vi "from string.vi"(8 "error in":errorcluster, 9 "data":string, 10 "version":string, 11 "Missing Plugin configuration in":refnum<class "Missing Plugin configuration.lvclass">) -> (0 "error out":errorcluster, 3 "Missing Plugin configuration out":refnum<class "Missing Plugin configuration.lvclass">)   [LabVIEW 2014, in "Missing Plugin configuration.lvclass"]
doc: "Provides an interface for loading a module configuration from a file or other serialized data source. It is recommended that all children of this class store data in two sets--data required for its own initialization, and any data required for parent initialization--and that each implementation uses the <b>Call Parent Method</b> primitive to de-serialize parent information. As a result, it is expected that every module configuration class calls <b>component configuration.lvclass:From String.vi</b>."
uses:
  Missing Plugin configuration.lvclass
  <vilib>/NI/Configuration Framework/serializable configuration/set view class name.vi
  <vilib>/NI/Tag Bus Module Framework/module configuration/TBM module configuration.lvclass
  <vilib>/NI/Configuration Framework/serializable configuration/NISE_CEF_serializable configuration.lvclass
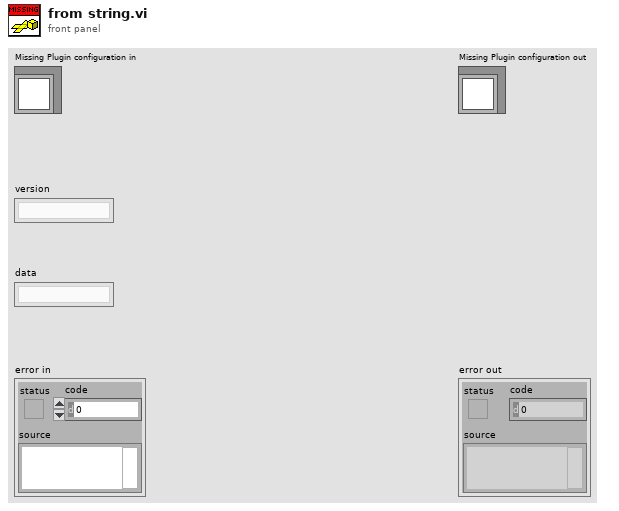
[diagram p1: front panel]
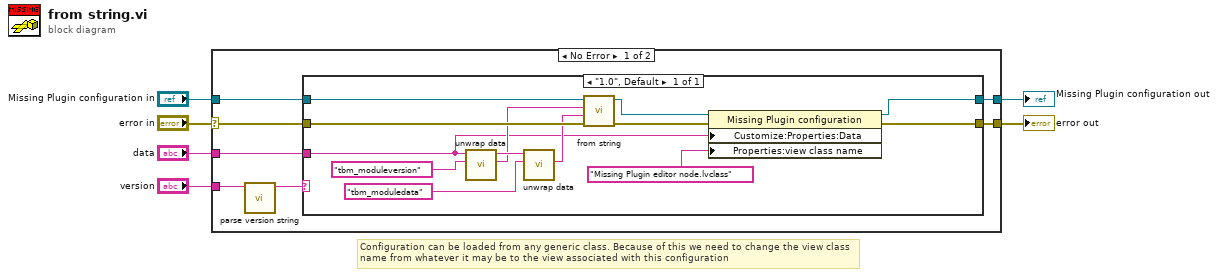
[diagram p0: block diagram]
diagram:
  # "Configuration can be loaded from any generic class. Because of this we need to change the view class name from whatever it may be to the view associated with this configuration"
  n1 = case shown="No Error" "error in" {
    selector: "error in" -> [w7 w28]
    tunnel: "data" -> [w13 _]
    tunnel: "Missing Plugin configuration in" -> [w12 w27]
    tunnel: [w11 w27] -> w5
    tunnel: [w10 w28] -> w4
    tunnel: "version" -> [w9 _]
    frame No Error {
      n2 = call <vilib>:"parse version string.vi"("full version"=w9) -> ("major.minor version"=w8:string)  [unwired: 7 in, 3 out]
      n3 = case shown="\"1.0\", Default" w8 {
        tunnel: w13 -> [w15]
        tunnel: w7 -> [w24]
        tunnel: w12 -> [w26]
        tunnel: [w16] -> w11
        tunnel: [w18] -> w10
        frame "1.0", Default {
          n4 = call <vilib>:"unwrap data.vi"("identifier"="tbm_moduleversion" ("additional identifier"), "data to unwrap"=w15) -> ("unwrapped data"=w20:string, "remaining string"=w25:string)  [unwired: 8 in]
          n5 = call <vilib>:"unwrap data.vi"("identifier"="tbm_moduledata" ("additional identifier"), "data to unwrap"=w25) -> ("unwrapped data"=w22:string)  [unwired: 8 in, 1 out]
          n6 = call-parent "from string.vi"("error in"=w24, "data"=w22, "version"=w20, "module configuration in"=w26) -> ("error out"=w19:errorcluster, "module configuration out"=w17:refnum<class "Missing Plugin configuration.lvclass">)  [unwired: 6 in]
          n7 = property class="Missing Plugin configuration"(reference=w17, error in=w19, "Customize:Properties:Data"=w15, "Properties:view class name"="Missing Plugin editor node.lvclass" ("view class name")) -> (reference out=w16:refnum<class "Missing Plugin configuration.lvclass">, error out=w18:errorcluster)
        }
      }
    }
    frame Error {
    }
  }
  "error out" <- w4
  "Missing Plugin configuration out" <- w5
